vi "OpenVariant Tree Example.vi"() -> ()   [LabVIEW 2013]
uses:
  source/Variant/OpenVariant.lvlib
panel:
  in  "Tree":string(tree)
  out "Variant Tree":variant
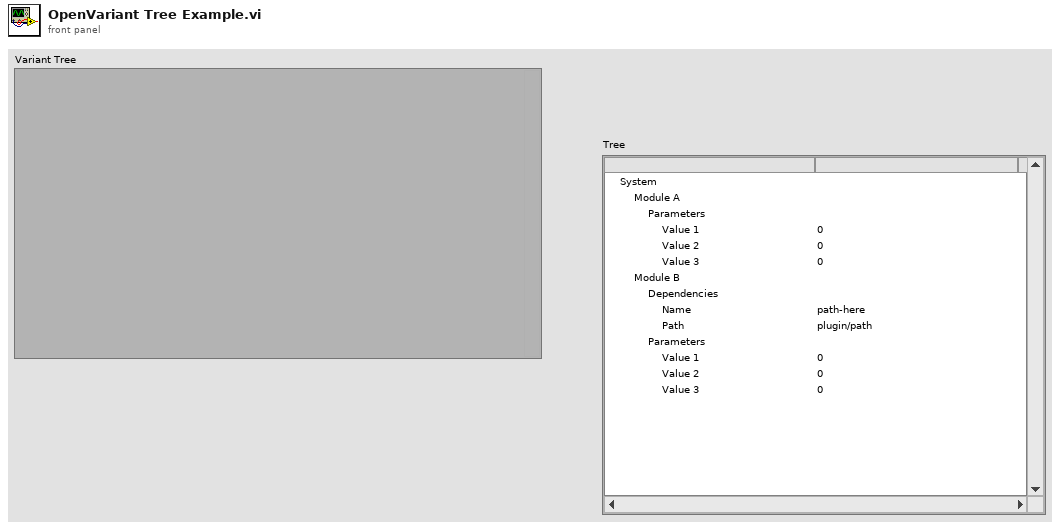
[diagram p1: front panel]
types:
  T1 = cluster{"Module A":cluster{"Parameters":cluster{"Value 1":dbl, "Value 2":dbl, "Value 3":dbl}}, "Module B":cluster{"Parameters":cluster{"Value 1":dbl, "Value 2":dbl, "Value 3":dbl}, "Dependencies":cluster{"Name":string, "Path":path}}}
  T2 = cluster{"Left Cell String":string, "Child Text":string[], "Child Tag":string, "Item Indent":i32, "Child Only?":bool, "Glyph Index":i32}[]
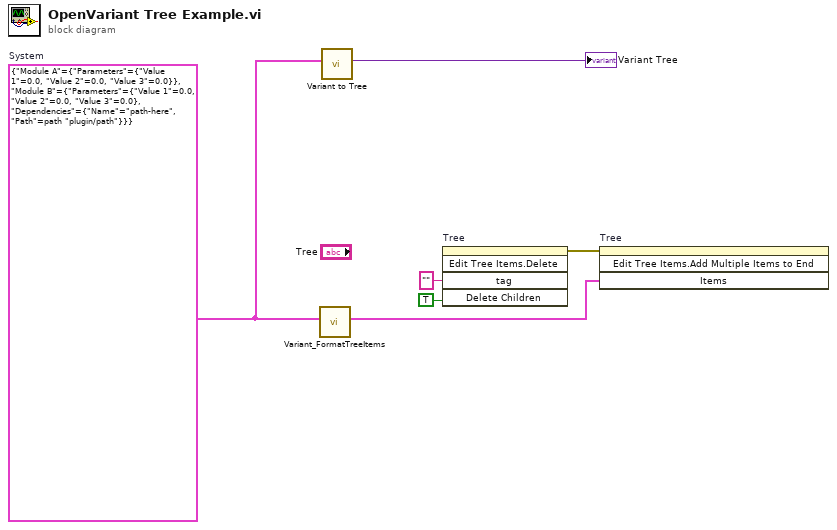
[diagram p0: block diagram]
diagram:
  w1 = T1 {"Module A"={"Parameters"={"Value 1"=0.0, "Value 2"=0.0, "Value 3"=0.0}}, "Module B"={"Parameters"={"Value 1"=0.0, "Value 2"=0.0, "Value 3"=0.0}, "Dependencies"={"Name"="path-here", "Path"=path "plugin/path"}}}  # System
  n1 = call "Variant_FormatTreeItems.vi"("Variant"=w1) -> ("Tree Items"=w5:T2)  [unwired: 10 in]
  n2 = call "Variant to Tree.vi"("Variant"=w1) -> ("Variant Tree"=→"Variant Tree":variant)  [unwired: 10 in]
  n3 = invoke on="Tree" class="Tree (strict)" method="Edit Tree Items.Delete"("tag"="" ("Tag"), "Delete Children"=TRUE ("Delete Children?")) -> (error out=w4:errorcluster)  [unwired: 3 in, 4 out]
  n4 = invoke on="Tree" class="Tree (strict)" method="Edit Tree Items.Add Multiple Items to End"(error in=w4, "Items"=w5) -> ()  [unwired: 2 in, 4 out]
